vi "Build VIH Deploy - List Files.vi"(6 "Exclude file names":string, 8 "error in":errorcluster, 9 "Exclude undesired paths (F)":bool, 10 "Folders":string, 11 "Source Dir":path) -> (0 "error out":errorcluster, 1 "Files to Copy":path[](array[path]), 2 "Project Files":path[](array[path]), 3 "dup Source Dir":path, 5 "Excluded Paths":path[](array[path]))   [LabVIEW 2014]
doc: "::: VI Helpeks :::\nCopyright (c) 2000-2026 Konstantin Shifershteyn. All rights reserved."
uses:
  <vilib>/Utility/lvfile.llb/NI_FileType.lvlib
panel:
  # "VI Helpeks\nCopyright (c) 2012-2026 Konstantin Shifershteyn"
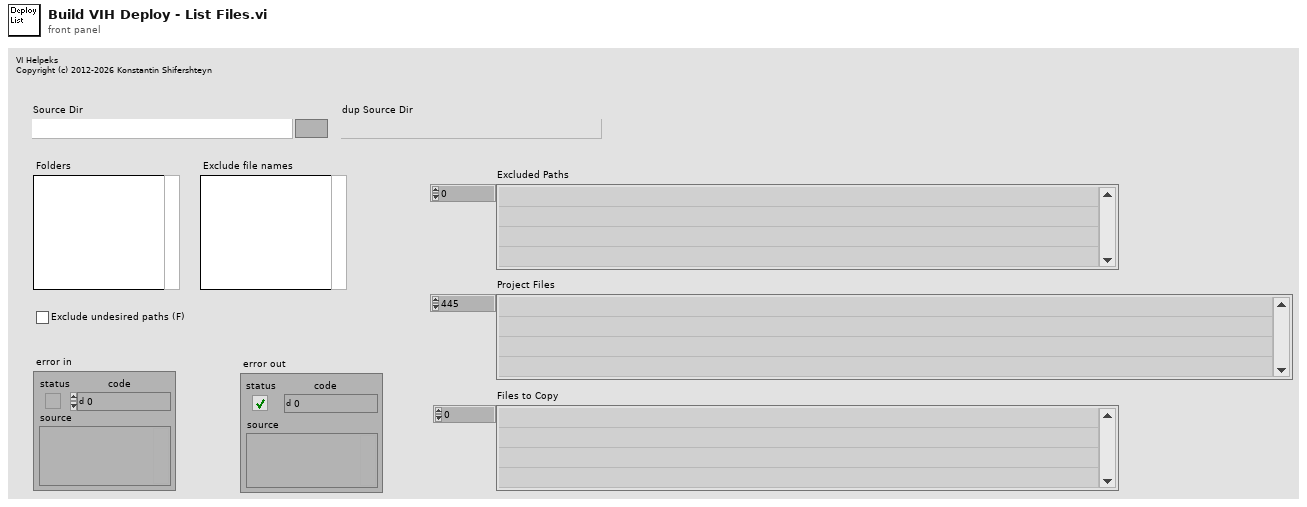
[diagram p1: front panel]
types:
  T1 = typedef "NI_FileType.lvlib/FT_FileTypes.ctl" = enum32{"Invalid file/path", "Unknown type", "Instrument", "Control", "Polymorphic VI", "Project", "Library", "LVClass", "XControl", "XNode", "CIN", "Run-time menu", "Palette menu", "LLB", "Shortcut", "Directory", "Class Private Data Control", "Statechart", "MathScript .m file", "Ladder Diagram", "LVLibp"}
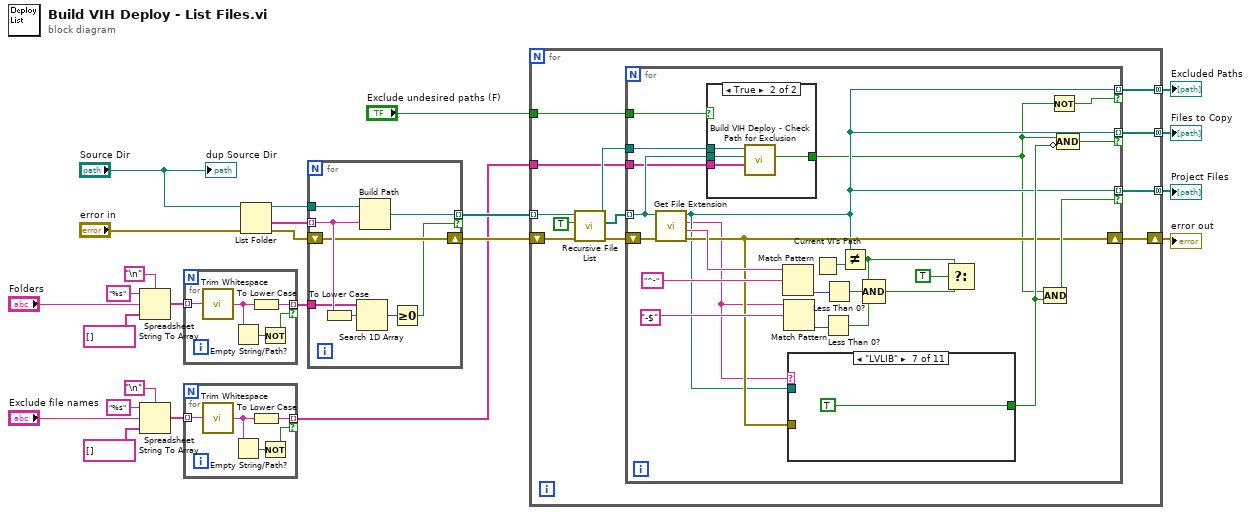
[diagram p0: block diagram]
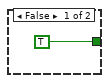
[diagram p2: hidden frame]
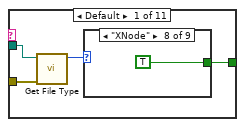
[diagram p3: hidden frame]
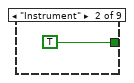
[diagram p5: hidden frame]
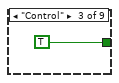
[diagram p6: hidden frame]
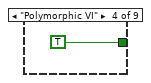
[diagram p7: hidden frame]
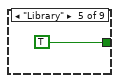
[diagram p8: hidden frame]
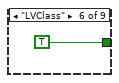
[diagram p9: hidden frame]
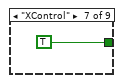
[diagram p10: hidden frame]
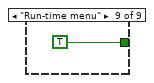
[diagram p11: hidden frame]
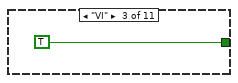
[diagram p13: hidden frame]
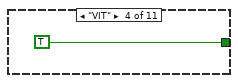
[diagram p14: hidden frame]
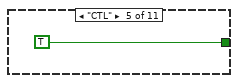
[diagram p15: hidden frame]
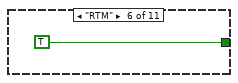
[diagram p16: hidden frame]
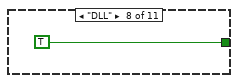
[diagram p17: hidden frame]
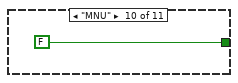
[diagram p19: hidden frame]
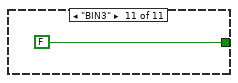
[diagram p20: hidden frame]
diagram:
  n1 = Spreadsheet String To Array(delimiter (Tab)="\n", format string="%s", spreadsheet string="Folders", array type (2D Dbl)=string[] []) -> (array=w7:string[])
  n2 = Spreadsheet String To Array(delimiter (Tab)="\n", format string="%s", spreadsheet string="Exclude file names", array type (2D Dbl)=string[] []) -> (array=w3:string[])
  n3 = for {
    tunnel: w7 -> [w29] mode=indexing
    tunnel: [w25] -> w22 mode=indexing if=w26
    n4 = call <vilib>:"Trim Whitespace.vi"("string"=w29) -> ("trimmed string"=w28:string)  [unwired: 1 in]
    n5 = Empty String/Path?(string/path=w28) -> (empty?=w27:bool)
    n6 = To Lower Case(string=w28) -> (all lower case string=w25:string)
    n7 = Not(x=w27) -> (.not. x?=w26:bool)
  }
  n8 = for {
    tunnel: w3 -> [w34] mode=indexing
    tunnel: [w30] -> w11 mode=indexing if=w31
    n9 = call <vilib>:"Trim Whitespace.vi"("string"=w34) -> ("trimmed string"=w33:string)  [unwired: 1 in]
    n10 = Empty String/Path?(string/path=w33) -> (empty?=w32:bool)
    n11 = To Lower Case(string=w33) -> (all lower case string=w30:string)
    n12 = Not(x=w32) -> (.not. x?=w31:bool)
  }
  n13 = List Folder(path="Source Dir", error in="error in") -> (path out=w21:path, folder names=w23:string[], error out=w19:errorcluster)  [unwired: 2 in, 1 out]
  n14 = for {
    tunnel: w23 -> [w41] mode=indexing
    tunnel: w22 -> [w35]
    tunnel: w21 -> [w42]
    tunnel: [w40] -> w20 mode=indexing if=w36
    shift-right: [w39] -> w18
    shift-left: w19 -> [w39]
    n15 = To Lower Case(string=w41) -> (all lower case string=w38:string)
    n16 = Search 1D Array(1D array=w35, element=w38) -> (index of element=w37:i32)  [unwired: 1 in]
    n17 = Build Path(base path=w42, name or relative path=w41) -> (appended path=w40:path)
    n18 = Greater Or Equal To 0?(x=w37) -> (x >= 0?=w36:bool)
  }
  n19 = for {
    tunnel: w20 -> [w51] mode=indexing
    shift-right: [w49] -> w15
    shift-left: w18 -> [w50]
    tunnel: [w48] -> w16 mode=concatenating
    tunnel: [w47] -> w17 mode=concatenating
    tunnel: "Exclude undesired paths (F)" -> [w45]
    tunnel: [w44] -> w12 mode=concatenating
    tunnel: w11 -> [w43]
    n20 = call <vilib>:"Recursive File List.vi"("error in (no error)"=w50, "Treat LLBs as Folders?"=TRUE, "Folder Path"=w51) -> ("error out"=w54:errorcluster, "All Files in Dir"=w52:path[], "dup Folder Path"=w46:path)  [unwired: 4 in, 2 out]
    n21 = for {
      tunnel: w52 -> [w62] mode=indexing
      tunnel: [w59] -> w48 mode=indexing if=w71
      shift-right: [w66] -> w49
      shift-left: w54 -> [w70]
      tunnel: [w59] -> w47 mode=indexing if=w67
      tunnel: w46 -> [w61]
      tunnel: w45 -> [w60]
      tunnel: [w59] -> w44 mode=indexing if=w57
      tunnel: w43 -> [w56]
      n22 = call <vilib>:"Get File Extension.vi"("error in (no error)"=w70, "file"=w62) -> ("error out"=w66:errorcluster, "filename without extension"=w78:string, "lowercase file extension"=w55:string, "dup file"=w59:path)  [unwired: 6 in]
      n23 = case shown="True" w60 {
        tunnel: w62 -> [_ w83]
        tunnel: w61 -> [_ w82]
        tunnel: [TRUE w81] -> w58
        tunnel: w56 -> [_ w80]
        frame False {
        }
        frame True {
          n24 = call "Build VIH Deploy - Check Path for Exclusion.vi"("Exclude file name patterns"=w80, "Path"=w83, "Base dir"=w82) -> ("pass"=w81:bool)  [unwired: 8 in]
        }
      }
      n25 = Match Pattern(string=w78, regular expression="^-") -> (offset past match=w75:i32)  [unwired: 1 in, 3 out]
      n26 = Match Pattern(string=w55, regular expression="-$") -> (offset past match=w76:i32)  [unwired: 1 in, 3 out]
      n27 = case shown="\"LVLIB\"" w55 {
        tunnel: [w85 _ TRUE TRUE TRUE TRUE TRUE TRUE _ FALSE FALSE] -> w68
        tunnel: w59 -> [w87 _ _ _ _ _ _ _ _ _ _]
        tunnel: w66 -> [w84 _ _ _ _ _ _ _ _ _ _]
        frame Default {
          n28 = call <vilib>:"Get File Type.vi"("error in (no error)"=w84, "path"=w87) -> ("file type"=w86:T1)  [unwired: 7 in, 2 out]
          n29 = case shown="\"XNode\"" w86 {
            tunnel: [_ TRUE TRUE TRUE TRUE TRUE TRUE TRUE TRUE] -> w85
            frame Default {
            }
            frame "Instrument" {
            }
            frame "Control" {
            }
            frame "Polymorphic VI" {
            }
            frame "Library" {
            }
            frame "LVClass" {
            }
            frame "XControl" {
            }
            frame "XNode" {
            }
            frame "Run-time menu" {
            }
          }
        }
        frame "----- 1" {
        }
        frame "VI" {
        }
        frame "VIT" {
        }
        frame "CTL" {
        }
        frame "RTM" {
        }
        frame "LVLIB" {
        }
        frame "DLL" {
        }
        frame "----- 2" {
        }
        frame "MNU" {
        }
        frame "BIN3" {
        }
      }
      n30 = Current VI's Path() -> (path=w69:path)
      n31 = Less Than 0?(x=w76) -> (x < 0?=w72:bool)
      n32 = Less Than 0?(x=w75) -> (x < 0?=w73:bool)
      n33 = Not Equal?(x=w59, y=w69) -> (x != y?=w65:bool)
      n34 = Compound Arithmetic op=AND(w65, w73, w72) -> (w64:bool)
      n35 = Select(t=w65, s=TRUE, f=w64) -> ()  [unwired: 1 out]
      n36 = Compound Arithmetic op=AND(w58, w68) -> (w71:bool)
      n37 = Not(x=w58) -> (.not. x?=w57:bool)
      n38 = Compound Arithmetic op=AND(w58, invert w68) -> (w67:bool)
    }
  }
  "error out" <- w15
  "Project Files" <- w16
  "Files to Copy" <- w17
  "Excluded Paths" <- w12
  "dup Source Dir" <- "Source Dir"
